vi "Release Tag Lock_ByRef.vi"(8 "error in (no error)":errorcluster, 9 "LockName":string, 10 "Tag Ref in":refnum<data-value>) -> (0 "error out":errorcluster, 2 "Tag Ref out":refnum<data-value>)   [LabVIEW 2020, in "Tag Engine.lvlib"]
doc: "Removes the lock LockName from the Tag given by reference. The Tag is unlocked when no locks remain."
uses:
  Tag Engine.lvlib
  Tag/Tag.lvclass
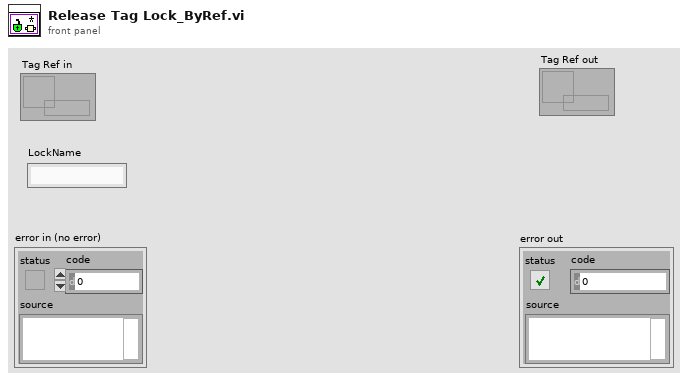
[diagram p1: front panel]
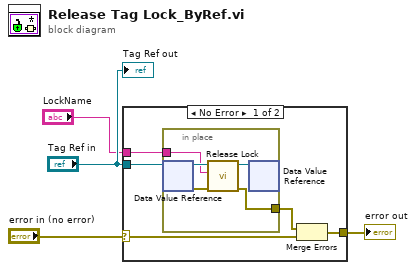
[diagram p0: block diagram]
diagram:
  n1 = case shown="No Error" "error in (no error)" {
    selector: "error in (no error)" -> [w8 w15]
    tunnel: "Tag Ref in" -> [w9 _]
    tunnel: [w7 w15] -> w4
    tunnel: "LockName" -> [w5 _]
    frame No Error {
      n2 = in-place {
        in-place-border: [w11] -> w6
        in-place-border: w5 -> [w12]
        n3 = in-place-dvr #1(w9) -> (w14:refnum<class "Tag.lvclass">, w10:errorcluster)
        n4 = call "Release Lock.vi"("error in (no error)"=w10, "LockName"=w12, "Tag in"=w14) -> ("error out"=w11:errorcluster, "Tag out"=w13:refnum<class "Tag.lvclass">)  [unwired: 7 in]
        n5 = in-place-dvr #1(w13) -> ()  [unwired: 2 out]
      }
      n6 = Merge Errors(w6, w8) -> (w7:errorcluster)
    }
    frame Error {
    }
  }
  "error out" <- w4
  "Tag Ref out" <- "Tag Ref in"
